vi "Lookup Sensor Scale.vi"(7 "SensorList":refnum<class "SensorList.lvclass">, 8 "error in (no error)":errorcluster, 11 "Scale in":refnum<class "Scale Config.lvclass">) -> (0 "error out":errorcluster, 2 "Sensor Scale":refnum<class "Scale Config.lvclass">, 3 "Scale out":refnum<class "Scale Config.lvclass">)   [LabVIEW 2020, in "VolatusConfig.lvlib" / "Scale Config.lvclass"]
uses:
  Scale Config.lvclass
  C:/dev/lv20CE/relink/lv-volatus/VolatusConfig/VolatusConfigElement/VolatusConfigElement.lvclass
  SensorList/SensorList.lvclass
  VolatusConfigElement/VolatusConfigElement.lvclass/VolatusConfigElement.ctl
  Meta Type.ctl
  VolatusConfigElement/Element.vi
  lv-cdm/CDM-Config/Config Element/Lookup Child by Name.vi
  lv-cdm/CDM-Config/Config Lookup/Match Meta.vi
  lv-cdm/CDM-Config/Config Element/Owner.vi
  lv-cdm/CDM-Config/Config Manager/Lookup Descendant.vi
  lv-cdm/CDM-Config/Config Filter/Config Lookup.lvclass
  Scale Config.lvclass/Scale Config.ctl
  VolatusConfigElement/VolatusConfigElement.lvclass
  VolatusConfig.lvlib
  lv-cdm/CDM-Config/Config Element/Config Element.lvclass
  Sensor/Sensor Config.lvclass
  C:/dev/lv20CE/relink/lv-volatus/VolatusConfig/Scale/Scale Config.lvclass
  C:/dev/lv20CE/relink/lv-volatus/VolatusConfig/SensorList/SensorList.lvclass
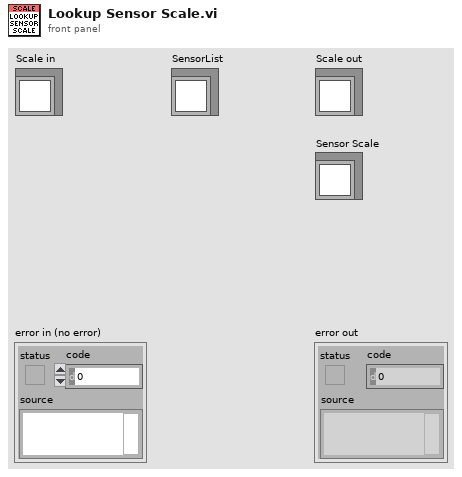
[diagram p1: front panel]
types:
  T1 = typedef "VolatusConfig.lvlib/Meta Type.ctl" = enum16{"UNKNOWN", "VL_System", "VL_Cluster", "VL_Node", "VL_Task", "VL_Group", "VL_Channel", "VL_Task_List", "VL_Scaling", "VL_Sensor", "VL_Sensor_List", "VL_Scale"}
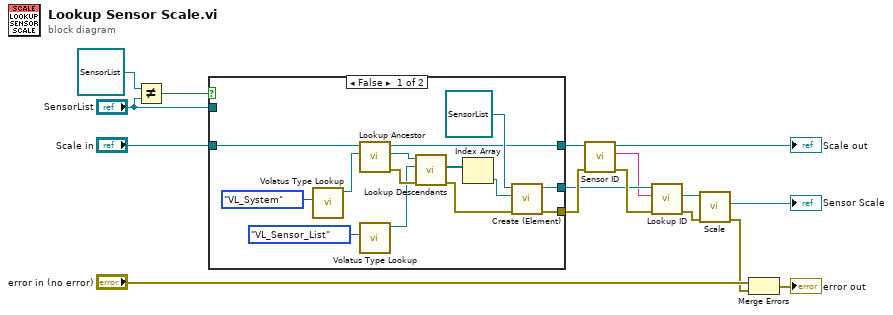
[diagram p0: block diagram]
diagram:
  n1 = Not Equal?(x=refnum<class "SensorList.lvclass"> refnum, y="SensorList") -> (x != y?=w6:bool)
  n2 = case shown="False" w6 {
    tunnel: [w22 w31] -> w4
    tunnel: [w21 w32] -> w14
    tunnel: "SensorList" -> [_ w32]
    tunnel: [w19 _] -> w15
    tunnel: "Scale in" -> [w17 w31]
    frame False {
      n3 = call "Volatus Type Lookup.vi"("Meta Type"=Meta_Type."VL_System") -> ("Config Lookup out"=w29:refnum<class "Config Lookup.lvclass">)  [unwired: 9 in, 1 out]
      n4 = call "Lookup Ancestor.vi"("Lookup"=w29, "VolatusConfigElement in"=w17) -> ("error out"=w30:errorcluster, "Ancestor"=w27:refnum<class "Config Element.lvclass">, "VolatusConfigElement out"=w22:refnum<class "Scale Config.lvclass">)  [unwired: 7 in]
      n5 = call "Volatus Type Lookup.vi"("Meta Type"=Meta_Type."VL_Sensor_List") -> ("Config Lookup out"=w25:refnum<class "Config Lookup.lvclass">)  [unwired: 9 in, 1 out]
      n6 = call "Lookup Descendants.vi"("error in (no error)"=w30, "Lookup"=w25, "Config Element in"=w27) -> ("error out"=w20:errorcluster, "Descendants"=w24:refnum<class "Config Element.lvclass">[])  [unwired: 6 in, 1 out]
      n7 = Index Array(array=w24) -> (element=w18:refnum<class "Config Element.lvclass">)  [unwired: 1 in]
      n8 = call "Create (Element).vi"("error in (no error)"=w20, "Element"=w18, "VolatusConfigElement in"=refnum<class "SensorList.lvclass"> refnum ("VolatusConfig.lvlib:SensorList.lvclass")) -> ("error out"=w19:errorcluster, "VolatusConfigElement out"=w21:refnum<class "SensorList.lvclass">)  [unwired: 7 in]
    }
    frame True {
    }
  }
  n9 = call "Sensor ID.vi"("error in (no error)"=w15, "Scale in"=w4) -> ("error out"=w16:errorcluster, "Sensor ID"=w2:string, "Scale out"=→"Scale out":refnum<class "Scale Config.lvclass">)  [unwired: 7 in]
  n10 = call "Lookup ID.vi"("error in (no error)"=w16, "ID"=w2, "SensorList in"=w14) -> ("error out"=w12:errorcluster, "Sensor"=w13:refnum<class "Sensor Config.lvclass">)  [unwired: 6 in, 1 out]
  n11 = call "Scale.vi"("error in (no error)"=w12, "Sensor in"=w13) -> ("error out"=w9:errorcluster, "Sensor Scale"=→"Sensor Scale":refnum<class "Scale Config.lvclass">)  [unwired: 7 in, 1 out]
  n12 = Merge Errors("error in (no error)", w9) -> (→"error out":errorcluster)
